vi "Parse Set Filter.vi"(8 "error in (no error)":errorcluster caption="에러 입력(에러 없음)", 10 "JSON string":string, 11 "Instrument Manager 입력":refnum<class "Instrument Manager.lvclass">) -> (0 "error out":errorcluster caption="에러 출력", 1 "Filter path":T1, 2 "Set Filter Param":T2, 3 "Instrument Manager 출력":refnum<class "Instrument Manager.lvclass">)   [LabVIEW 2023, in "Instrument Manager.lvclass"]
uses:
  Instrument Manager.lvclass
  Param Definition/Set Filter Path Param.ctl
  Module/CE RF Switch Box/Type Definition/Filter path.ctl
  Instrument Manager.lvclass/Instrument Manager.ctl
  Module/CE RF Switch Box/RF Switch Box.lvlib
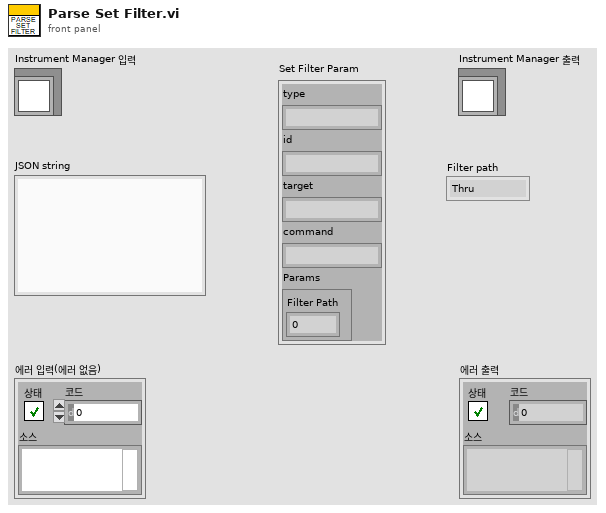
[diagram p1: front panel]
types:
  T1 = typedef "RF Switch Box.lvlib/Filter path.ctl" = enum16{"Thru", "Direct Amp", "1G HPF", "3G HPF", "7G HPF", "6G HPF", "port 1", "port 2", "port 3", "port 4", "port 5", "port 6", "port 7", "port 8", "port 9", "port 10", "port 11", "port 12", "port 13", "port 14", "port 15", "port 16", "port 17", "port 18"}
  T2 = typedef "Instrument Manager.lvclass/Set Filter Path Param.ctl" = cluster{"type":string, "id":string, "target":string, "command":string, "Params":cluster{"Filter Path":i32}}
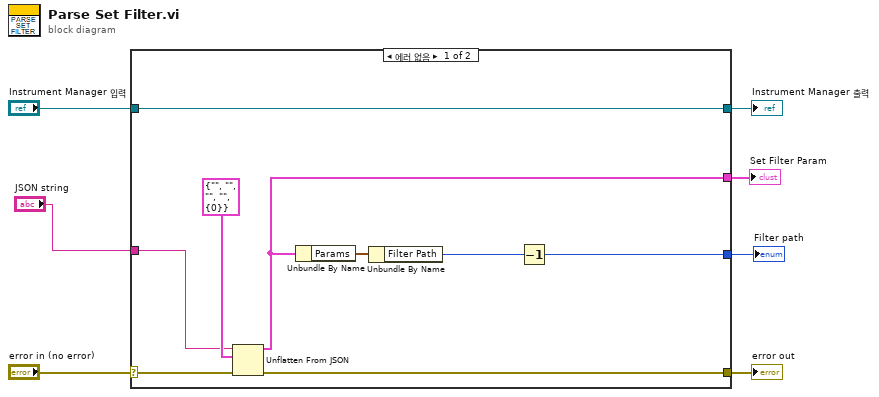
[diagram p0: block diagram]
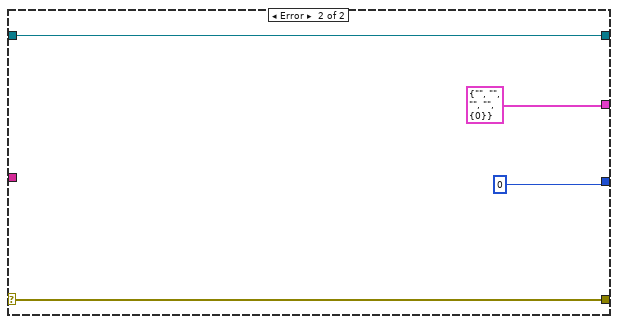
[diagram p2: hidden frame]
diagram:
  n1 = case shown="에러 없음" "error in (no error)" {
    selector: "error in (no error)" -> [w13 w20]
    tunnel: [w12 w20] -> w6
    tunnel: [w16 w19] -> w4
    tunnel: "Instrument Manager 입력" -> [w16 w19]
    tunnel: "JSON string" -> [w14 _]
    tunnel: [w11 T2 {"type"="", "id"="", "target"="", "command"="", "Params"={"Filter Path"=0}} ("Set Filter Param")] -> w2
    tunnel: [w8 0 ("Filter Path")] -> w1
    frame No Error {
      n2 = Unflatten From JSON(JSON string=w14, type and defaults=T2 {"type"="", "id"="", "target"="", "command"="", "Params"={"Filter Path"=0}} ("Set Filter Param"), error in (no error)=w13) -> (value=w11:T2, error out=w12:errorcluster)  [unwired: 4 in]
      n3 = Unbundle By Name(w11) -> ("Params"=w10:cluster{"Filter Path":i32})
      n4 = Unbundle By Name(w10) -> ("Filter Path"=w9:i32)
      n5 = Decrement(x=w9) -> (x-1=w8:i32)
    }
    frame Error {
    }
  }
  "error out" <- w6
  "Instrument Manager 출력" <- w4
  "Set Filter Param" <- w2
  "Filter path" <- w1
